vi "TsFile-9ch-VI-aligned-isolated.vi"() -> ()   [LabVIEW 2026]
uses:
  .tmp/TsFile-LabVIEW-9ch-Fair-2026-11-04/bin/x86/libtsfile_isol_vi.dll
panel:
  out "status (0 = OK)":i32
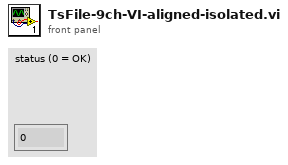
[diagram p1: front panel]
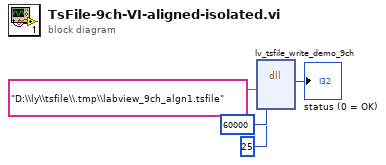
[diagram p0: block diagram]
diagram:
  n1 = dll-call lib="D:/ly/tsfile/.tmp/TsFile-LabVIEW-9ch-Fair-2026-11-04/bin/x86/libtsfile_isol_vi.dll" fn="lv_tsfile_write_demo_9ch"("tsfile_path"="D:\\ly\\tsfile\\.tmp\\labview_9ch_algn1.tsfile", "rows_per_block"=60000, "blocks"=25) -> ("return type"=→"status (0 = OK)":i32)  [unwired: 6 in, 2 out]
